vi "Enumerate EStop Sources.vi"() -> (7 "Implementation Map":T1(c390))   [LabVIEW 2025, in "VolatusControl.lvlib" / "EStop Module.lvclass"]
uses:
  EStop Module.lvclass
  EStop Module.lvclass/EStop Module.ctl
  EStop Source/EStop Source.lvclass
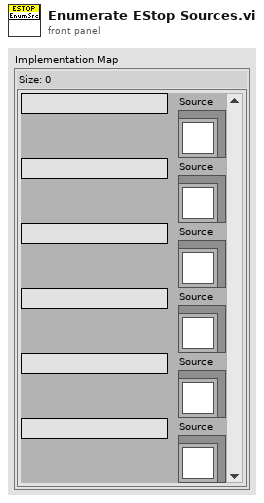
[diagram p1: front panel]
types:
  T1 = map{string, refnum<class "EStop Source.lvclass">}
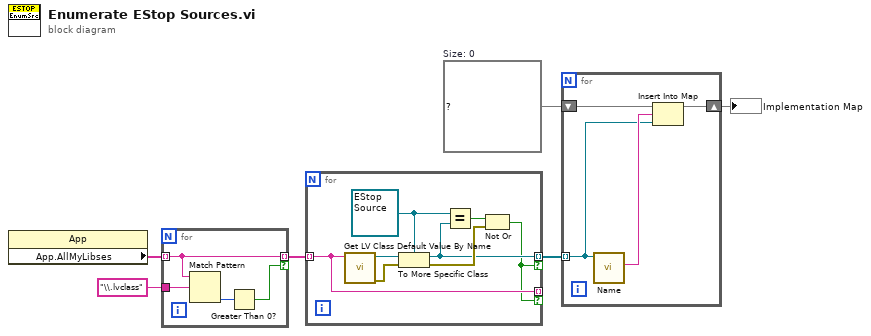
[diagram p0: block diagram]
diagram:
  w2 = T1 {}  # Size: 0
  n1 = property class="App"() -> ("App.AllMyLibses"=w6:string[])  [unwired: 2 in, 2 out]
  n2 = for {
    tunnel: w6 -> [w8] mode=indexing
    tunnel: "\\.lvclass" -> [w10]
    tunnel: [w8] -> w4 mode=indexing if=w7
    n3 = Match Pattern(string=w8, regular expression=w10) -> (offset past match=w9:i32)  [unwired: 1 in, 3 out]
    n4 = Greater Than 0?(x=w9) -> (x > 0?=w7:bool)
  }
  n5 = for {
    tunnel: w4 -> [w12] mode=indexing
    tunnel: [w13] -> w3 mode=indexing if=w11
    tunnel: [w12] -> _ mode=indexing if=w11
    w17 = refnum<class "EStop Source.lvclass"> refnum ("VolatusControl.lvlib:EStop Source.lvclass")
    n6 = call <vilib>:"Get LV Class Default Value By Name.vi"("class name"=w12) -> ("error out"=w16:errorcluster, "object"=w18:refnum<class>)  [unwired: 9 in]
    n7 = To More Specific Class(target class=w17, reference=w18, error in=w16) -> (specific class reference=w13:refnum<class "EStop Source.lvclass">, error out=w15:errorcluster)
    n8 = Equal?(x=w17, y=w13) -> (x = y?=w14:bool)
    n9 = Not Or(1:w15, 2:w14) -> (0:w11:bool)
  }
  n10 = for {
    tunnel: w3 -> [w20] mode=indexing
    shift-right: [w19] -> w1
    shift-left: w2 -> [w22]
    n11 = call-dynamic "Name.vi"("EStop Source in"=w20) -> ("Name"=w21:string)  [unwired: 10 in]
    n12 = Insert Into Map(map in=w22, key=w21, value=w20) -> (map out=w19:T1)  [unwired: 2 out]
  }
  "Implementation Map" <- w1
